vi "apply_gamma_planar.vi"(8 "error in (no error)":errorcluster, 10 "gamma_value":sgl=0.9, 11 "image in":T1) -> (0 "error out":errorcluster, 3 "image out":T1)   [LabVIEW 2017, in "Image Processing Library.lvlib"]
uses:
  Image Processing Library.lvlib
  <vilib>/picture/picture.llb/imagedata.ctl
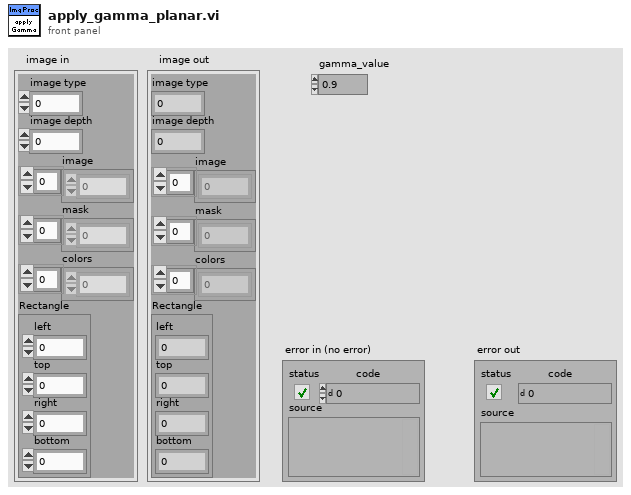
[diagram p1: front panel]
types:
  T1 = typedef "imagedata.ctl" = cluster{"image type":i32, "image depth":i32, "image":u8[], "mask":u8[], "colors":u32[], "Rectangle":cluster{"left":i16, "top":i16, "right":i16, "bottom":i16}}
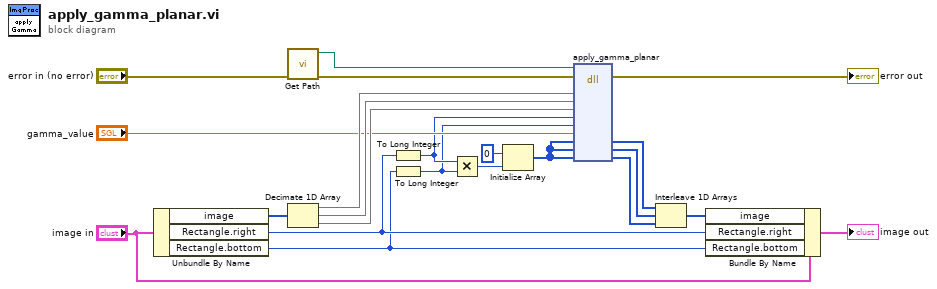
[diagram p0: block diagram]
diagram:
  n1 = Unbundle By Name("image in") -> ("image"=w18:u8[], "Rectangle.right"=w2:i16, "Rectangle.bottom"=w1:i16)
  n2 = call "Get Path.vi"("error in (no error)"="error in (no error)") -> ("error out"=w21:errorcluster, "Library Path"=w20:path)  [unwired: 9 in]
  n3 = Decimate 1D Array(w18) -> (w17:u8[], w16:u8[], w15:u8[])
  n4 = To Long Integer(number=w2) -> (32bit integer=w4:i32)
  n5 = To Long Integer(number=w1) -> (32bit integer=w3:i32)
  n6 = Multiply(x=w4, y=w3) -> (x*y=w5:i32)
  n7 = Initialize Array(u8 0 ("element"), w5) -> (w6:u8[])
  n8 = dll-call lib="C:/Users/IvanLis-Win10/Desktop/LabVIEW/Coin Detector/Project_2018/image_processing/windows_x64/image_processing.dll" fn="apply_gamma_planar"(path in=w20, error in=w21, "in_r"=w17, "in_g"=w16, "in_b"=w15, "orig_w"=w4, "orig_h"=w3, "gamma_value"="gamma_value", "out_r"=w6, "out_g"=w6, "out_b"=w6) -> (error out=→"error out":errorcluster, "out_r"=w14:u8[], "out_g"=w13:u8[], "out_b"=w12:u8[])  [unwired: 8 in, 1 out]
  n9 = Interleave 1D Arrays(w14, w13, w12) -> (w11:u8[])
  n10 = Bundle By Name(cluster="image in", "image"=w11, "Rectangle.right"=w2, "Rectangle.bottom"=w1) -> (→"image out":T1)
